vi "Pose3d_Exp.vi"(9 "Twist3d":T1, 11 "Pose3d":T2={"Translation3d"={"X"=0.0, "Y"=0.0, "Z"=0.0}, "Rotation3d"={"Q_quaternion"={"R"=1.0, "V"=[0.0, 0.0, 0.0]}}} {"Translation3d"."Z" format="%14.3f"; "Translation3d"."Y" format="%14.3f"; "Translation3d"."X" format="%14.3f"}) -> (0 "Error":bool, 3 "Updated Pose3d":T2={"Translation3d"={"X"=0.0, "Y"=0.0, "Z"=0.0}, "Rotation3d"={"Q_quaternion"={"R"=1.0, "V"=[0.0, 0.0, 0.0]}}} {"Translation3d"."Z" format="%14.3f"; "Translation3d"."Y" format="%14.3f"; "Translation3d"."X" format="%14.3f"})   [LabVIEW 2019, in "Trajectory_Library.lvlib"]
doc: "Obtain a new Pose3d from a (constant curvature) velocity.\n\nThe twist is a change in pose in the robot's coordinate frame since the previous pose update. When the user runs exp() on the previous known field-relative pose with the argument being the twist, the user will receive the new field-relative pose.\n\n\"Exp\" represents the pose exponential, which is solving a differential equation moving the pose forward in time. Obtain a new Pose2d from a (constant curvature) velocity.\n\n\nPARAMETERS:\n--------------\n - POSE3D - current POSE data structure\n - TWIST 3D- TThe change in pose in the robot's coordinate frame since the previous pose update. For example, if a non-holonomic robot moves forward 0.01 meters and changes angle by 0.5 degrees since the previous pose update, the twist would be Twist3d(0.01, 0.0, 0.0, new new Rotation3d(0.0, 0.0, Units.degreesToRadians(0.5))).\n\nRETURNS:\n-----------\n- OUT POSE3D - The new pose of the robot.\n- Error -- boolean -- If TRUE, an error occured."
uses:
  Trajectory_Library.lvlib
  TypeDef/POSE3D.ctl
  TypeDef/TRANSLATION3D.ctl
  TypeDef/ROTATION3D.ctl
  TypeDef/QUATERNION.ctl
  TypeDef/TWIST3D.ctl
  <vilib>/Analysis/baseanly.llb/Real A x B.vi
  MatBuilder_Fill.vi
  Pose3d_TransformBy.vi
  MatBuilder_Create.vi
  <vilib>/Analysis/7linalg.llb/Matrix Power.vi
  <vilib>/Analysis/7linalg.llb/Real Matrix Power.vi
  <vilib>/Analysis/7linalg.llb/Matrix Exp.vi
  <vilib>/Analysis/7linalg.llb/Real Matrix Exp.vi
  Quaternion_New.vi
  Rotation3d_Create_Quaternion.vi
  Matrix_Transpose.vi
  <vilib>/Analysis/baseanly.llb/Determinant.vi
  <vilib>/Analysis/baseanly.llb/Real Determinant.vi
  Matrix_NormF.vi
  Pose3d_getTranslation3d.vi
  Pose3d_getRotation3d.vi
  Transform3d_GetTranslation3d.vi
  Transform3d_GetRotation3d.vi
  Translation3d_Plus.vi
  Translation3d_RotateBy.vi
  Pose3d_New_Trans3dRot3d.vi
  Rotation3d_Plus.vi
  Quaternion_Normalize.vi
  <vilib>/Analysis/_algsub.llb/Matrix Norm.vi
  <vilib>/Analysis/_algsub.llb/Real Matrix Norm.vi
  Rotation3d_GetQuaterion.vi
  Quaternion_Times.vi
  Quaternion_Inverse.vi
  Quaternion_Get_All.vi
  Rotation3d_RotateBy.vi
  Quaternion_New_Default.vi
  <vilib>/Analysis/7linalg.llb/Create Special Matrix.vi
  <vilib>/Analysis/7linalg.llb/Create Special Real Matrix.vi
  <vilib>/Analysis/7linalg.llb/Matrix Logarithm.vi
  <vilib>/Analysis/7linalg.llb/Real Matrix Logarithm.vi
  <vilib>/Analysis/Matrix/Numeric/Complex/Complex To Cartesian.vi
  <vilib>/Analysis/Matrix/Numeric/Complex/Complex To Cartesian - CM.vi
  <vilib>/Analysis/Matrix/Numeric/Multiply/Multiply - RM,R.vi
  <vilib>/Analysis/Matrix/Numeric/Add/Add - RM,RM.vi
  <vilib>/Analysis/Matrix/Numeric/Subtract/Subtract.vi
  <vilib>/Analysis/Matrix/Numeric/Subtract/Subtract - RM,RM.vi
  <vilib>/Analysis/NI_AALBase.lvlib
  <vilib>/Analysis/Matrix/NI_Matrix.lvlib
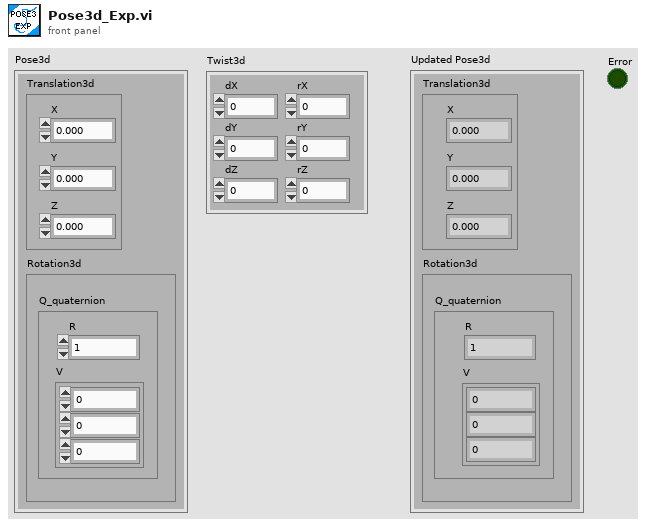
[diagram p1: front panel]
types:
  T1 = typedef "Trajectory_Library.lvlib/TWIST3D.ctl" = cluster{"dX":dbl, "dY":dbl, "dZ":dbl, "rX":dbl, "rY":dbl, "rZ":dbl}
  T2 = typedef "Trajectory_Library.lvlib/POSE3D.ctl" = cluster{"Translation3d":T3, "Rotation3d":T4}
  T3 = typedef "Trajectory_Library.lvlib/TRANSLATION3D.ctl" = cluster{"X":dbl, "Y":dbl, "Z":dbl}
  T4 = typedef "Trajectory_Library.lvlib/ROTATION3D.ctl" = cluster{"Q_quaternion":T5}
  T5 = typedef "Trajectory_Library.lvlib/QUATERNION.ctl" = cluster{"R":dbl, "V":dbl[]}
  T6 = typedef "NI_Matrix.lvlib/RealMatrix.ctl" = dbl[][]
  T7 = typedef "Trajectory_Library.lvlib/TRANSFORM3D.ctl" = cluster{"TRANSLATION3D":T3, "ROTATION3D":T4, "XF":bool}
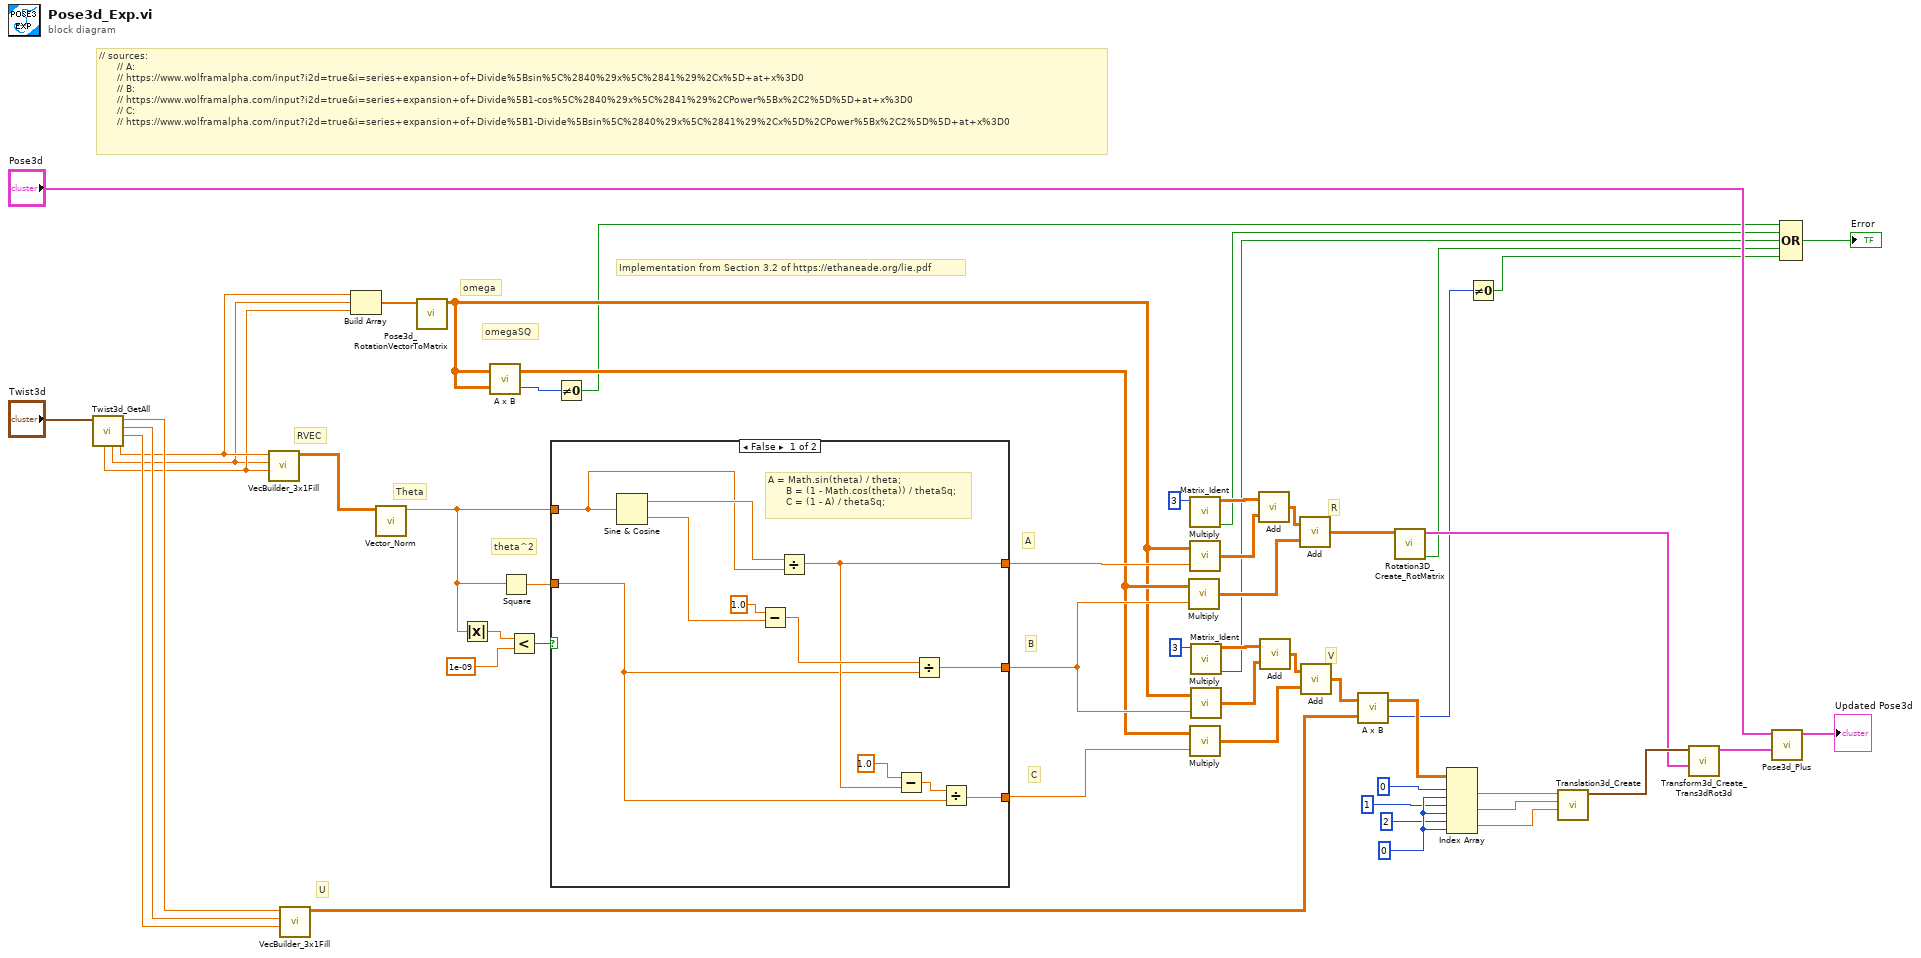
[diagram p0: block diagram]
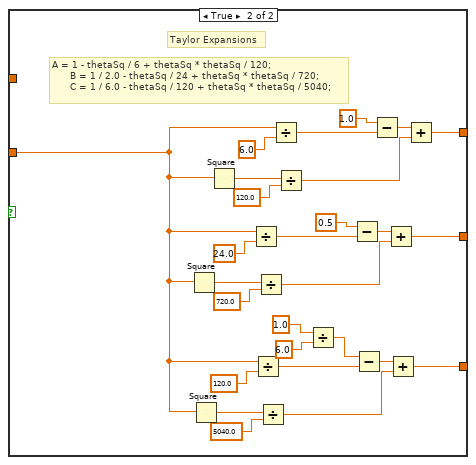
[diagram p2: hidden frame]
diagram:
  w12 = 0 ("index (col)")
  # "// sources:\n      // A:\n      // https://www.wolframalpha.com/input?i2d=true&i=series+expansion+of+Divide%5Bsin%5C%2840%29x%5C%2841%29%2Cx%5D+at+x%3D0\n      // B:\n      // https://www.wolframalpha.com/input?i2d=true&i=series+expansion+of+Divide%5B1-cos%5C%2840%29x%5C%2841%29%2CPower%5Bx%2C2%5D%5D+at+x%3D0\n      // C:\n      // https://www.wolframalpha.com/input?i2d=true&i=series+expansion+of+Divide%5B1-Divide%5Bsin%5C%2840%29x%5C%2841%29%2Cx%5D%2CPower%5Bx%2C2%5D%5D+at+x%3D0"
  # "V"
  # "R"
  # "Implementation from Section 3.2 of https://ethaneade.org/lie.pdf"
  # "C"
  # "B"
  # "A"
  # "Theta"
  # "omegaSQ"
  # "RVEC"
  # "U"
  # "theta^2"
  # "omega"
  n1 = call "Twist3d_GetAll.vi"("Twist3d"="Twist3d") -> ("rX"=w44:dbl, "dZ"=w45:dbl, "dY"=w46:dbl, "dX"=w47:dbl, "rY"=w38:dbl, "rZ"=w43:dbl)  [unwired: 5 in]
  n2 = call "VecBuilder_3x1Fill.vi"("R2"=w43, "R1"=w38, "R0"=w44) -> ("output matrix"=w40:T6)  [unwired: 8 in]
  n3 = call "VecBuilder_3x1Fill.vi"("R2"=w45, "R1"=w46, "R0"=w47) -> ("output matrix"=w22:T6)  [unwired: 8 in]
  n4 = Build Array(w44, w38, w43) -> (w42:dbl[])
  n5 = call "Vector_Norm.vi"("Input Vector"=w40) -> ("norm"=w1:dbl)  [unwired: 10 in]
  n6 = call "Pose3d_RotationVectorToMatrix.vi"("RotationVector"=w42) -> ("Rotation Matrix"=w5:T6)  [unwired: 10 in]
  n7 = Absolute Value(x=w1) -> (abs(x)=w2:dbl)
  n8 = call-poly <vilib>:"A x B.vi"("B"=w5, "A"=w5) -> ("error"=w4:i32, "A x B"=w6:T6)
  n9 = Square(x=w1) -> (x^2=w39:dbl)
  n10 = Less?(x=w2, y=1e-09) -> (x < y?=w53:bool)
  n11 = case shown="False" w53 {
    tunnel: w39 -> [w55 w66]
    tunnel: [w56 w84] -> w35
    tunnel: [w58 w67] -> w25
    tunnel: [w54 w65] -> w24
    tunnel: w1 -> [w61 _]
    frame False {
      # "A = Math.sin(theta) / theta;\n      B = (1 - Math.cos(theta)) / thetaSq;\n      C = (1 - A) / thetaSq;"
      n12 = Sine & Cosine(0:w61) -> (1:w62:dbl, 2:w60:dbl)
      n13 = Subtract(x=1.0, y=w60) -> (x-y=w59:dbl)
      n14 = Divide(x=w62, y=w61) -> (x/y=w56:dbl)
      n15 = Subtract(x=1.0, y=w56) -> (x-y=w63:dbl)
      n16 = Divide(x=w59, y=w55) -> (x/y=w58:dbl)
      n17 = Divide(x=w63, y=w55) -> (x/y=w54:dbl)
    }
    frame True {
      # "A = 1 - thetaSq / 6 + thetaSq * thetaSq / 120;\n      B = 1 / 2.0 - thetaSq / 24 + thetaSq * thetaSq / 720;\n      C = 1 / 6.0 - thetaSq / 120 + thetaSq * thetaSq / 5040;"
      # "Taylor Expansions"
      n18 = Square(x=w66) -> (x^2=w77:dbl)
      n19 = Square(x=w66) -> (x^2=w71:dbl)
      n20 = Square(x=w66) -> (x^2=w85:dbl)
      n21 = Divide(x=w66, y=24.0) -> (x/y=w79:dbl)
      n22 = Divide(x=w66, y=120.0) -> (x/y=w73:dbl)
      n23 = Divide(x=w77, y=720.0) -> (x/y=w78:dbl)
      n24 = Divide(x=w71, y=5040.0) -> (x/y=w72:dbl)
      n25 = Divide(x=w66, y=6.0) -> (x/y=w87:dbl)
      n26 = Divide(x=w85, y=120.0) -> (x/y=w86:dbl)
      n27 = Divide(x=1.0, y=6.0) -> (x/y=w68:dbl)
      n28 = Subtract(x=0.5, y=w79) -> (x-y=w82:dbl)
      n29 = Subtract(x=w68, y=w73) -> (x-y=w76:dbl)
      n30 = Subtract(x=1.0, y=w87) -> (x-y=w90:dbl)
      n31 = Add(x=w82, y=w78) -> (x+y=w67:dbl)
      n32 = Add(x=w76, y=w72) -> (x+y=w65:dbl)
      n33 = Add(x=w90, y=w86) -> (x+y=w84:dbl)
    }
  }
  n34 = Not Equal To 0?(x=w4) -> (x != 0?=w3:bool)
  n35 = call-poly <vilib>:"Multiply.vi"("Real Scalar c"=w25, "Real Matrix A"=w6) -> ("A * c"=w31:T6)
  n36 = call "Matrix_Ident.vi"("Size"=3) -> ("Error"=w21:bool, "output matrix"=w34:T6)  [unwired: 9 in]
  n37 = call-poly <vilib>:"Multiply.vi"("Real Scalar c"=w35, "Real Matrix A"=w5) -> ("A * c"=w32:T6)
  n38 = call-poly <vilib>:"Multiply.vi"("Real Scalar c"=w24, "Real Matrix A"=w6) -> ("A * c"=w26:T6)
  n39 = call "Matrix_Ident.vi"("Size"=3) -> ("Error"=w20:bool, "output matrix"=w29:T6)  [unwired: 9 in]
  n40 = call-poly <vilib>:"Multiply.vi"("Real Scalar c"=w25, "Real Matrix A"=w5) -> ("A * c"=w27:T6)
  n41 = call-poly <vilib>:"Add.vi"("Real Matrix B"=w32, "Real Matrix A"=w34) -> ("A + B"=w33:T6)
  n42 = call-poly <vilib>:"Add.vi"("Real Matrix B"=w27, "Real Matrix A"=w29) -> ("A + B"=w28:T6)
  n43 = call-poly <vilib>:"Add.vi"("Real Matrix B"=w31, "Real Matrix A"=w33) -> ("A + B"=w18:T6)
  n44 = call-poly <vilib>:"Add.vi"("Real Matrix B"=w26, "Real Matrix A"=w28) -> ("A + B"=w23:T6)
  n45 = call-poly <vilib>:"A x B.vi"("B"=w22, "A"=w23) -> ("error"=w15:i32, "A x B"=w19:T6)
  n46 = call "Rotation3D_Create_RotMatrix.vi"("RotationMatrix"=w18) -> ("Error"=w16:bool, "Rotation3d"=w17:T4)  [unwired: 9 in]
  n47 = Index Array(array=w19, index (row) #1=0 ("index (row)"), index (col) #1=w12, index (row) #2=1 ("index (row)"), index (col) #2=w12, index (row) #3=2 ("index (row)"), index (col) #3=w12) -> (element #1=w9:dbl, element #2=w8:dbl, element #3=w7:dbl)
  n48 = Not Equal To 0?(x=w15) -> (x != 0?=w14:bool)
  n49 = call "Translation3d_Create.vi"("Z"=w7, "Y"=w8, "X"=w9) -> ("TRANSLATION3D"=w51:T3)  [unwired: 8 in]
  n50 = call "Transform3d_Create_Trans3dRot3d.vi"("Rotation3d"=w17, "Translation3d"=w51) -> ("Transform3d"=w50:T7)  [unwired: 9 in]
  n51 = call "Pose3d_Plus.vi"("other Transform3d"=w50, "in Pose3d"="Pose3d") -> ("out Pose3d"=→"Updated Pose3d":T2)  [unwired: 9 in]
  n52 = Compound Arithmetic op=OR(w3, w21, w20, w16, w14) -> (→"Error":bool)
